vi "Test_C_W12_W13_W14_W15.vi"() -> ()   [LabVIEW 2021]
uses:
  CANsub_C.lvlib
  C_Decode_Result.ctl
panel:
  out "encode frame":u8[](array[numeric]) format="%.0x"
  out "W15 len":i32
  out "length":i32
  out "echo frame":u8[](array[numeric]) format="%.0x"
  out "size data":i32
  out "id":u32[](array[numeric]) format="%.0x"
  out "data len":u8[](array[numeric])
  out "dlc":u8[](array[numeric])
  out "size hdlc":i32
  out "size ping":i32
  out "data":u8[](array[numeric])
  out "size ws":i32
  out "result":T1
  # "Expected values when run."
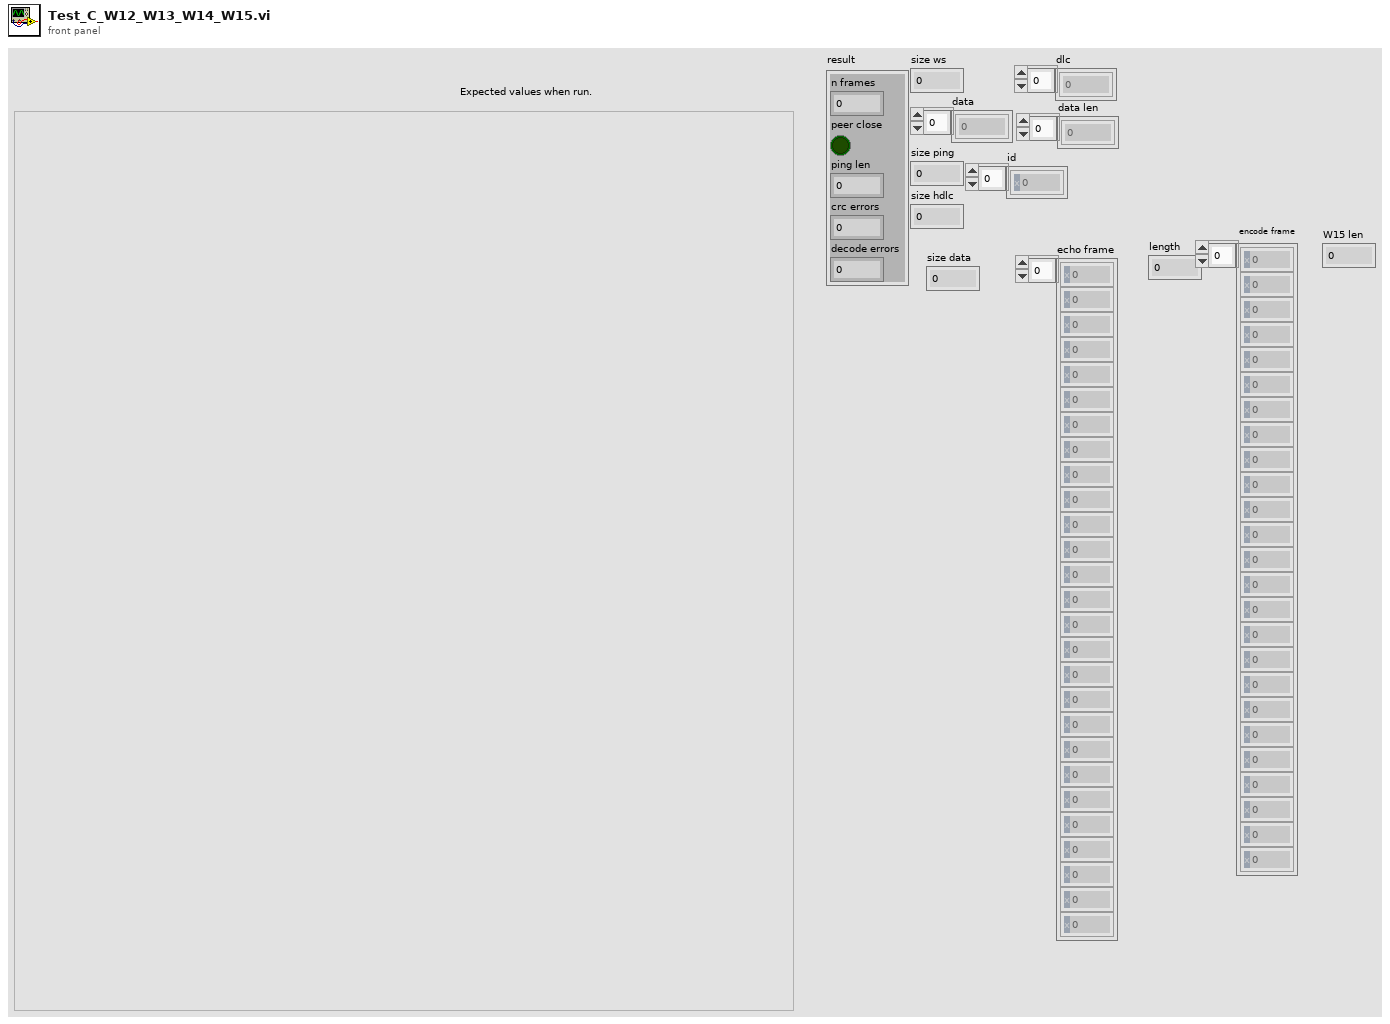
[diagram p1: front panel]
types:
  T1 = typedef "CANsub_C.lvlib/C_Decode_Result.ctl" = cluster{"n frames":i32, "peer close":bool, "ping len":i32, "crc errors":u32, "decode errors":i32}
  T2 = typedef "CANsub_C.lvlib/C_RX_Buffers.ctl" = cluster{"t_dev":dbl[], "ws":u8[], "id":u32[], "flags":u16[], "hdlc":u8[], "dlc":u8[], "data len":u8[], "data":u8[], "ping":u8[]}
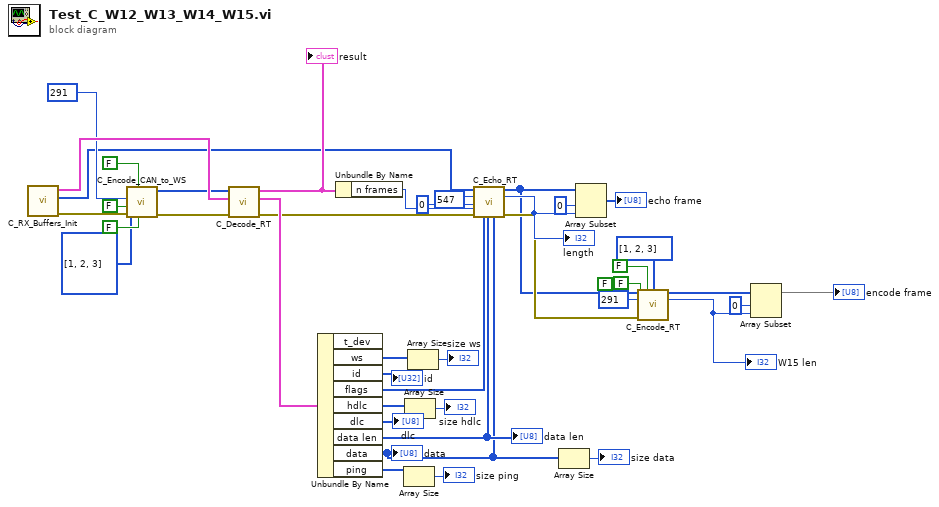
[diagram p0: block diagram]
diagram:
  n1 = call "C_RX_Buffers_Init.vi"() -> ("error out"=w41:errorcluster, "tx"=w12:u8[], "buffers"=w39:T2)  [unwired: 8 in, 1 out]
  n2 = call "C_Encode_CAN_to_WS.vi"("brs"=FALSE, "ide"=FALSE, "error in (no error)"=w41, "fdf"=FALSE, "id"=u32 291, "data"=u8[] [1, 2, 3]) -> ("error out"=w40:errorcluster, "ws frame"=w19:u8[])  [unwired: 4 in]
  n3 = call "C_Decode_RT.vi"("error in (no error)"=w40, "buffers in"=w39, "bytes in"=w19) -> ("error out"=w24:errorcluster, "buffers out"=w42:T2, "result"=w21:T1)  [unwired: 6 in]
  "result" <- w21
  n4 = Unbundle By Name(w42) -> ("ws"=w33:u8[], "id"=→"id":u32[], "flags"=w18:u16[], "hdlc"=w29:u8[], "dlc"=→"dlc":u8[], "data len"=w17:u8[], "data"=w16:u8[], "ping"=w31:u8[])  [unwired: 1 out]
  "data" <- w16
  "data len" <- w17
  n5 = Unbundle By Name(w21) -> ("n frames"=w20:i32)
  n6 = Array Size(array=w31) -> (size(s)=→"size ping":i32)
  n7 = Array Size(array=w29) -> (size(s)=→"size hdlc":i32)
  n8 = Array Size(array=w33) -> (size(s)=→"size ws":i32)
  n9 = call "C_Echo_RT.vi"("tx in"=w12, "flags"=w18, "data len"=w17, "data"=w16, "new id"=u32 547, "index"=0, "n frames"=w20, "error in (no error)"=w24) -> ("tx out"=w5:u8[], "length"=w15:i32, "error out"=w11:errorcluster)  [unwired: 5 in]
  "length" <- w15
  n10 = Array Size(array=w16) -> (size(s)=→"size data":i32)
  n11 = Array Subset(array=w5, index=0, length=w15) -> (→"echo frame":u8[])
  n12 = call "C_Encode_RT.vi"("tx in"=w5, "brs"=FALSE, "data"=u8[] [1, 2, 3], "id"=u32 291, "ide"=FALSE, "fdf"=FALSE, "error in (no error)"=w11) -> ("tx out"=w4:u8[], "length"=w2:i32)  [unwired: 6 in, 1 out]
  "W15 len" <- w2
  n13 = Array Subset(array=w4, index=0, length=w2) -> (→"encode frame":u8[])
